vi "Func - Get list of numeric arguments.vi"(5 "InstanceRef":T1, 6 "error in":bool, 7 "max arg num":i32=100, 8 "min arg num":i32=1, 9 "arg list":T2[](array[typedef])) -> (0 "error out":bool, 3 "val list":dbl[](array[numeric]))   [LabVIEW 2021]
doc: "This VI returns the values of function arguments which must all have the <b>DBL Number</b> data type. It verifies the number of actual arguments and their data types. Refer to the VI help for more details.\n\n<b>arg list</b> specifies the list of function arguments passed to a FuncVI. Wire it to the same terminal on the FuncVI block diagram.\n\n<b>min arg num</b> and <b>max arg num</b> specify the minimum and the maximum number of arguments allowed.\n\n::: CalcExpress Toolkit :::\nCopyright (c) 2000-2026 Konstantin Shifershteyn. All rights reserved."
uses:
  cetypes.llb/CalcExpress Function Argument Info.ctl
  cetypes.llb/CalcExpress Instance RefNum.ctl
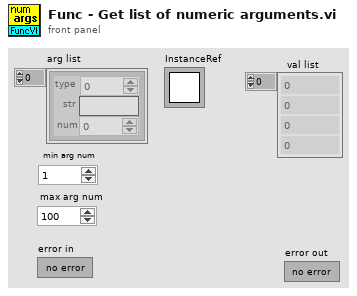
[diagram p1: front panel]
types:
  T1 = typedef "CalcExpress Instance RefNum.ctl" = refnum<k1>
  T2 = typedef "CalcExpress Function Argument Info.ctl" = cluster{"type":u32, "str":string, "num":dbl}
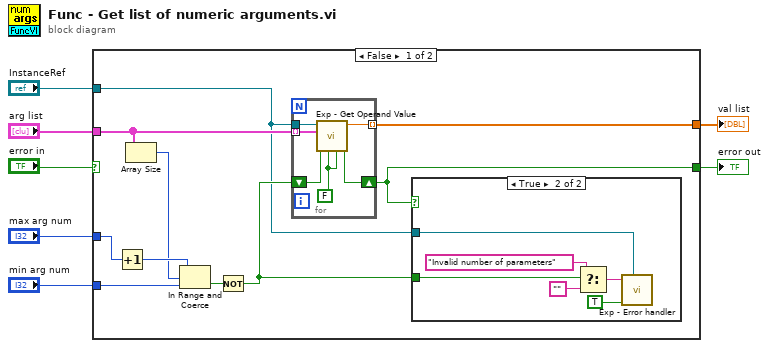
[diagram p0: block diagram]
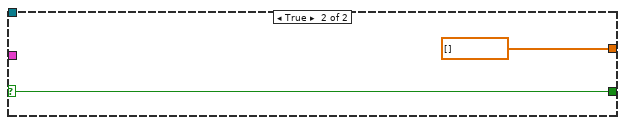
[diagram p3: hidden frame]
diagram:
  n1 = case shown="False" "error in" {
    selector: "error in" -> [_ w30]
    tunnel: [w13 dbl[] []] -> w7
    tunnel: [w12 w30] -> w6
    tunnel: "arg list" -> [w11 _]
    tunnel: "InstanceRef" -> [w8 _]
    tunnel: "max arg num" -> [w10 _]
    tunnel: "min arg num" -> [w9 _]
    frame False {
      n2 = Increment(x=w10) -> (x+1=w16:i32)
      n3 = Array Size(array=w11) -> (size(s)=w15:i32)
      n4 = In Range and Coerce(upper limit=w16, x=w15, lower limit=w9) -> (In Range?=w14:bool)  [unwired: 1 out]
      n5 = Not(x=w14) -> (.not. x?=w17:bool)
      n6 = for {
        tunnel: w11 -> [w20] mode=indexing
        shift-right: [w22] -> w12
        shift-left: w17 -> [w23]
        tunnel: [w21] -> w13 mode=indexing
        tunnel: w8 -> [w19]
        w18 = FALSE ("may be string ? (F)")
        n7 = call "Exp - Get Operand Value.vi"("ena complex? (F)"=w18, "ena string? (F)"=w18, "error in"=w23, "op info"=w20, "InstanceRef"=w19) -> ("error out"=w22:bool, "num"=w21:dbl)  [unwired: 1 in, 2 out]
      }
      n8 = case shown="True" w12 {
        tunnel: w17 -> [_ w29]
        tunnel: w8 -> [_ w24]
        frame False {
        }
        frame True {
          n9 = Select(t="Invalid number of parameters" ("ErrStr"), s=w29, f="" ("Empty String Constant")) -> (s? t:f=w25:string)
          n10 = call "Exp - Error handler.vi"("InstanceRef"=w24, "error in"=TRUE, "error message in"=w25) -> ()  [unwired: 6 in, 3 out]
        }
      }
    }
    frame True {
    }
  }
  "error out" <- w6
  "val list" <- w7
